vi "Variant Type is sortable.vi"(8 "error in (no error)":errorcluster, 11 "Type":variant) -> (0 "error out":errorcluster, 3 "Sortable ?":bool)   [LabVIEW 2012, in "Scripting Tools.lvlib" / "XNode Support.lvlib"]
uses:
  XNode Support.lvlib
  <vilib>/Utility/VariantDataType/VariantType.lvlib
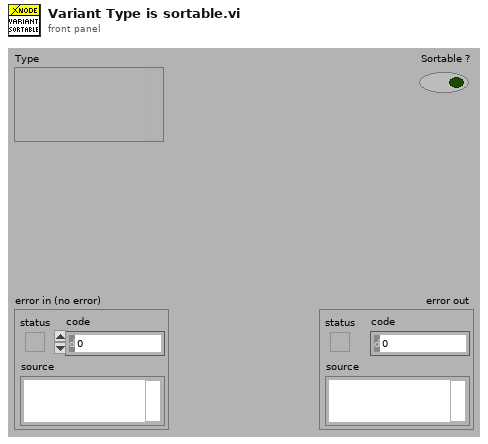
[diagram p1: front panel]
types:
  T1 = typedef "VariantType.lvlib/Type.ctl" = enum8{"Invalid Type", "Void", "I8", "I16", "I32", "I64", "U8", "U16", "U32", "U64", "Single Float", "Double Float", "Extended Float", "Single Complex", "Double Complex", "Extended Complex", "Enum U8", "Enum U16", "Enum U32", "Enum U64", "Single Float With Unit", "Double Float With Unit", "Extended Float With Unit", "Single Complex with Unit", "Double Complex with Unit", "Extended Complex with Unit", "Boolean", "String", "Path", "Picture", "Tag", "Array", "Cluster", "Variant", "LV Variant", "Waveform", "Timestamp", "Digital Waveform", "Digital Data", "ExpressData", "Refnum", "External Data", "VI", "Poly VI", "LabVIEW Class Instance", "Fixed Point"}
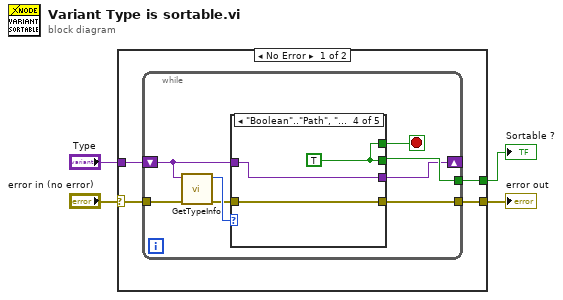
[diagram p0: block diagram]
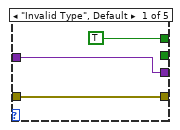
[diagram p2: hidden frame]
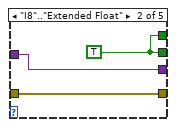
[diagram p3: hidden frame]
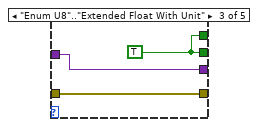
[diagram p4: hidden frame]
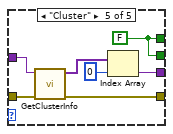
[diagram p5: hidden frame]
diagram:
  n1 = case shown="No Error" "error in (no error)" {
    selector: "error in (no error)" -> [w5 w36]
    tunnel: "Type" -> [w8 _]
    tunnel: [w7 _] -> w3
    tunnel: [w6 w36] -> w2
    frame No Error {
      n2 = while {
        tunnel: [w16] -> w7
        tunnel: [w10] -> w6
        tunnel: w5 -> [w14]
        shift-right: [w12] -> _
        shift-left: w8 -> [w13]
        stop <- w9 stop-if-true
        n3 = call <vilib>:"GetTypeInfo.vi"("error in (no error)"=w14, "Variant"=w13) -> ("error out"=w11:errorcluster, "Type Enum"=w15:T1)  [unwired: 8 out]
        n4 = case shown="\"Boolean\"..\"Path\", \"Timestamp\"" w15 {
          tunnel: [_ w20 w23 w26 w35] -> w16
          tunnel: w13 -> [w19 w22 w25 w28 w34]
          tunnel: [w19 w22 w25 w28 w29] -> w12
          tunnel: w11 -> [w18 w21 w24 w27 w33]
          tunnel: [w18 w21 w24 w27 w32] -> w10
          tunnel: [TRUE w20 w23 w26 w35] -> w9
          frame "Invalid Type", Default {
          }
          frame "I8".."Extended Float" {
            w20 = TRUE
          }
          frame "Enum U8".."Extended Float With Unit" {
            w23 = TRUE
          }
          frame "Boolean".."Path", "Timestamp" {
            w26 = TRUE
          }
          frame "Cluster" {
            w35 = FALSE
            n5 = call <vilib>:"GetClusterInfo.vi"("error in (no error)"=w33, "Variant"=w34) -> ("error out"=w32:errorcluster, "Cluster Elements"=w31:variant[])  [unwired: 8 out]
            n6 = Index Array(array=w31, index=0) -> (element=w29:variant)
          }
        }
      }
    }
    frame Error {
    }
  }
  "Sortable ?" <- w3
  "error out" <- w2
